vi "CSM - Read INI String.vi"(4 "Write If not found? (F)":bool, 5 "Section Name (\"\" as Default)":string, 7 "error in (no error)":errorcluster, 8 "Default Value":string, 9 "Variable Name":string) -> (1 "error out":errorcluster, 2 "Key Found?":bool, 3 "Value":string)   [LabVIEW 2017, in "INI-Static-Variable-Support.lvlib"]
doc: "Reads the configuration information string. This VI retrieves the raw string description without replacing INI variable references.\n\n<b>Application Scenario</b>: Need to read raw configuration information instead of configuration information after replacing internal variable references.\n\n<b>Reference Example</b>: `6. Read Nested Variables.vi`.\n\n-- <b>Controls</b> --\n- <b>Section Name (\"\" as Default)</b>: Section name. An empty string indicates the default section.\n- <b>Key</b>: Input string containing variable references.\n- <b>Default Value</b>: Default value.\n- <b>Write If not found? (F)</b>: Whether to write the default value if not found.\n\n-- <b>Indicators</b> --\n- <b>Value</b>: Output string after replacing variables.\n- <b>Key Found?</b>: Whether the key exists."
uses:
  INI-Static-Variable-Support.lvlib
  _fgv-oper.ctl
  <userlib>/_NEVSTOP/Communicable State Machine(CSM)/_Support/ChangeFlag/ChangeFlag-Read.vi
  <userlib>/_NEVSTOP/Communicable State Machine(CSM)/_Support/ChangeFlag/ChangeFlagDB.vi
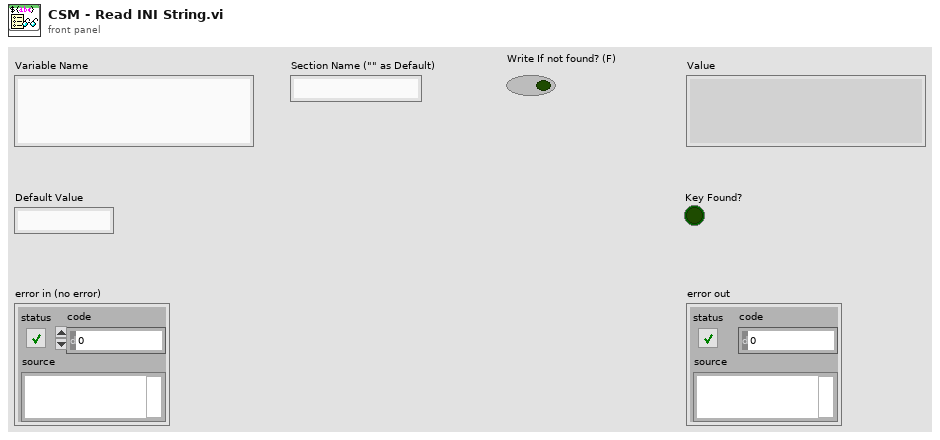
[diagram p1: front panel]
types:
  T1 = typedef "INI-Static-Variable-Support.lvlib/_fgv-oper.ctl" = enum16{"Read", "Write", "Sync", "Sessions", "List Keys", "Load", "List Files", "List Variables", "List Permanent Variables", "Mark Temp Variable as Permenent", "unload", "INIConfig(Memory)", "Reset", "Restore Variable Value"}
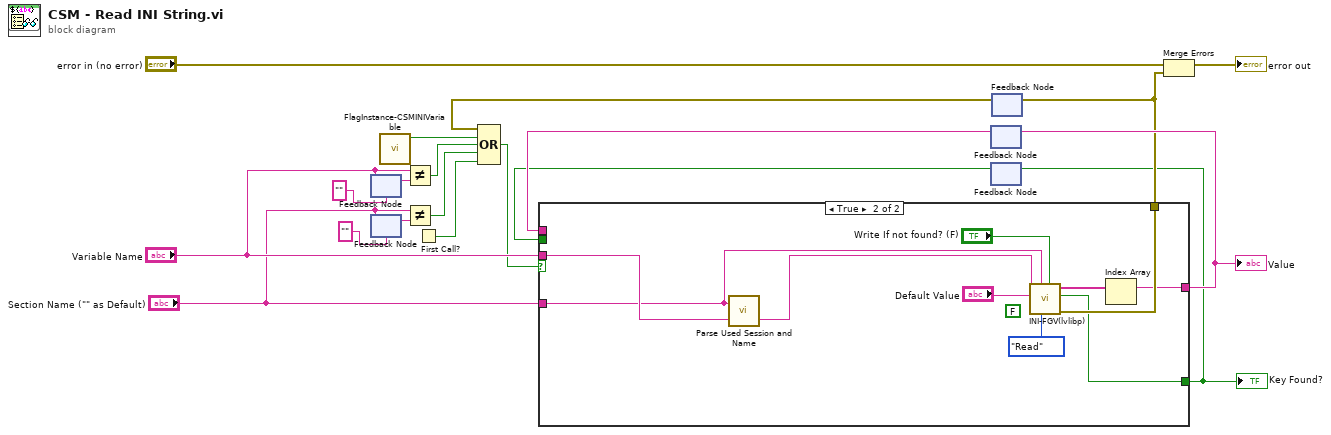
[diagram p0: block diagram]
diagram:
  n1 = feedback #1("") -> (w17:string)
  n2 = feedback-in #1("Variable Name") -> ()
  n3 = feedback #2("") -> (w16:string)
  n4 = feedback-in #2("Section Name (\"\" as Default)") -> ()
  n5 = call "FlagInstance-CSMINIVariable.vi"() -> ("Changed"=w1:bool)  [unwired: 10 in, 1 out]
  n6 = Not Equal?(x="Variable Name", y=w17) -> (x != y?=w13:bool)
  n7 = Not Equal?(x="Section Name (\"\" as Default)", y=w16) -> (x != y?=w12:bool)
  n8 = First Call?() -> (First Call?: T/F=w2:bool)
  n9 = feedback #3() -> (w10:string)  [unwired: 1 in]
  n10 = feedback #4() -> (w7:bool)  [unwired: 1 in]
  n11 = feedback #5() -> (w6:errorcluster)  [unwired: 1 in]
  n12 = Compound Arithmetic op=OR(w6, w1, w13, w12, w2) -> (w5:bool)
  n13 = case shown="True" w5 {
    tunnel: [_ w29] -> w9
    tunnel: [w21 w26] -> w11
    tunnel: [w20 w27] -> w8
    tunnel: "Variable Name" -> [_ w24]
    tunnel: "Section Name (\"\" as Default)" -> [_ w22]
    tunnel: w10 -> [w21 _]
    tunnel: w7 -> [w20 _]
    frame False {
    }
    frame True {
      (unwired) FALSE ("Raw String? (F)")
      n14 = call "Parse Used Session and Name.vi"("name"=w24, "Section Name(\"\" as Default)"=w22) -> ("used name"=w23:string)  [unwired: 1 in]
      n15 = call "INI-FGV(lvlibp).vi"("Write If not found?"="Write If not found? (F)", "Enum"=_fgv-oper."Read", "Prefered Section"=w22, ">> Default Value >>"="Default Value", ">> Variable Name >>"=w23) -> ("error out"=w29:errorcluster, "Key?"=w27:bool, "Array"=w28:string[])  [unwired: 3 in, 1 out]
      n16 = Index Array(array=w28) -> (element=w26:string)  [unwired: 1 in]
    }
  }
  "Value" <- w11
  "Key Found?" <- w8
  n17 = feedback-in #3(w11) -> ()
  n18 = feedback-in #4(w8) -> ()
  n19 = feedback-in #5(w9) -> ()
  n20 = Merge Errors("error in (no error)", w9) -> (→"error out":errorcluster)
